vi "Test Remove Project.vi"(8 "error in (no error)":errorcluster, 10 "Work Folder":path, 11 "Test Data Folder":path) -> (0 "error out":errorcluster, 2 "Report":string, 3 "Passed":bool)   [LabVIEW 2024]
doc: "Removes the sample project \"Client Website\" with Project Store-INI, writes, and reads the files again into a NEW store: the project and all its tasks must be gone from memory and from disk, and the other projects must still be there.\n\nInputs: Test Data Folder holds the source copies (Samples, v1); each run works in a new case folder under Work Folder. Passed is TRUE when every check passed and no error occurred; Report lists every check.\n\nGenerated by: Claude"
uses:
  Storage/Project Store-INI/Project Store-INI.lvclass
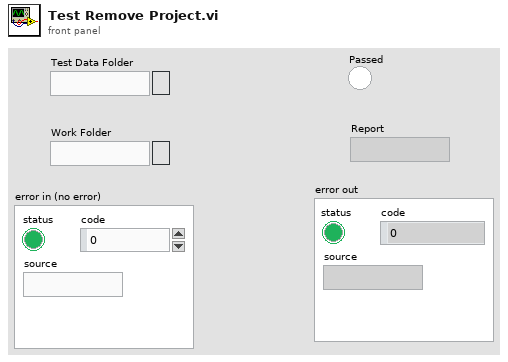
[diagram p1: front panel]
types:
  T1 = typedef "Task List.ctl" = T2[]
  T2 = typedef "Task.ctl" = cluster{"ID":string, "Project ID":string, "Name":string, "Active":bool, "Sort Order":i32}
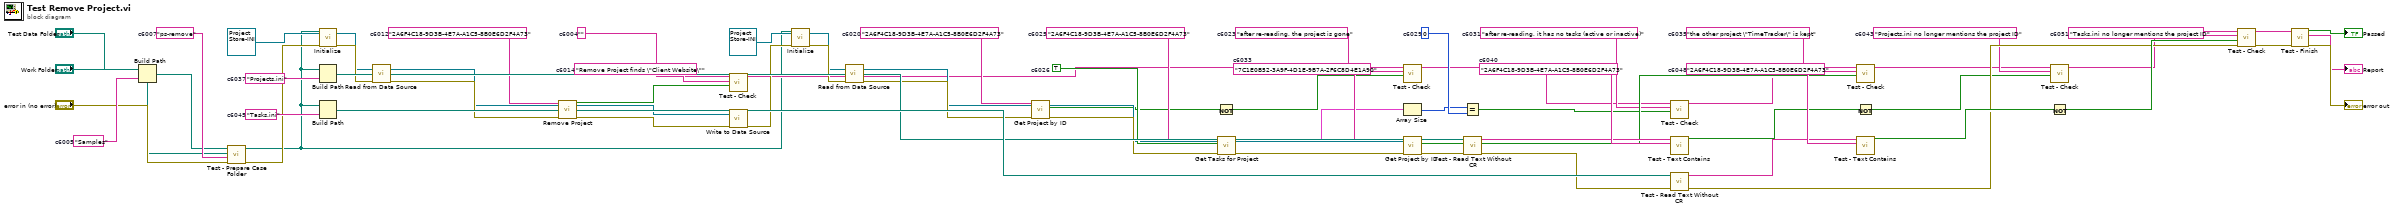
[diagram p0: block diagram]
diagram:
  w65 = "Tasks.ini no longer mentions the project ID"  # c6051
  w62 = "2A6F4C18-9D3B-4E7A-A1C5-8B0E6D2F4A73"  # c6048
  w58 = "Tasks.ini"  # c6045
  w56 = "Projects.ini no longer mentions the project ID"  # c6043
  w53 = "2A6F4C18-9D3B-4E7A-A1C5-8B0E6D2F4A73"  # c6040
  w49 = "Projects.ini"  # c6037
  w47 = "the other project \"TimeTracker\" is kept"  # c6035
  w44 = "7C1E0B52-3A9F-4D1E-9B7A-2F6C8D4E1A90"  # c6033
  w42 = "after re-reading, it has no tasks (active or inactive)"  # c6031
  w40 = 0  # c6029
  w35 = TRUE  # c6026
  w34 = "2A6F4C18-9D3B-4E7A-A1C5-8B0E6D2F4A73"  # c6025
  w32 = "after re-reading, the project is gone"  # c6023
  w27 = "2A6F4C18-9D3B-4E7A-A1C5-8B0E6D2F4A73"  # c6020
  w19 = "Remove Project finds \"Client Website\""  # c6014
  w15 = "2A6F4C18-9D3B-4E7A-A1C5-8B0E6D2F4A73"  # c6012
  w7 = "ps-remove"  # c6007
  w5 = "Samples"  # c6005
  w4 = ""  # c6004
  n1 = Build Path(base path="Test Data Folder", name or relative path=w5) -> (appended path=w6:path)
  n2 = call "Test - Prepare Case Folder.vi"("error in (no error)"="error in (no error)", "Case Name"=w7, "Work Folder"="Work Folder", "Source Folder"=w6) -> ("error out"=w9:errorcluster, "Case Folder"=w8:path)  [unwired: 6 in]
  n3 = call-dynamic "Initialize.vi"("Project Store in"=refnum<class "Project Store-INI.lvclass"> refnum ("Project Store-INI"), "error in (no error)"=w9, "Data Folder"=w8) -> ("error out"=w12:errorcluster, "Project Store out"=w11:refnum<class "Project Store-INI.lvclass">)  [unwired: 7 in]
  n4 = Build Path(base path=w8, name or relative path=w49) -> (appended path=w50:path)
  n5 = Build Path(base path=w8, name or relative path=w58) -> (appended path=w59:path)
  n6 = call-dynamic "Read from Data Source.vi"("Project Store in"=w11, "error in (no error)"=w12) -> ("error out"=w14:errorcluster, "Project Store out"=w13:refnum<class "Project Store-INI.lvclass">)  [unwired: 8 in]
  n7 = call-dynamic "Remove Project.vi"("Project Store in"=w13, "error in (no error)"=w14, "ID"=w15) -> ("error out"=w18:errorcluster, "found?"=w16:bool, "Project Store out"=w17:refnum<class "Project Store-INI.lvclass">)  [unwired: 6 in]
  n8 = call "Test - Check.vi"("Condition"=w16, "Check Name"=w19, "Report in"=w4) -> ("Report out"=w20:string)  [unwired: 7 in, 1 out]
  n9 = call-dynamic "Write to Data Source.vi"("Project Store in"=w17, "error in (no error)"=w18) -> ("error out"=w21:errorcluster)  [unwired: 8 in, 1 out]
  n10 = call-dynamic "Initialize.vi"("Project Store in"=refnum<class "Project Store-INI.lvclass"> refnum ("Project Store-INI"), "error in (no error)"=w21, "Data Folder"=w8) -> ("error out"=w24:errorcluster, "Project Store out"=w23:refnum<class "Project Store-INI.lvclass">)  [unwired: 7 in]
  n11 = call-dynamic "Read from Data Source.vi"("Project Store in"=w23, "error in (no error)"=w24) -> ("error out"=w26:errorcluster, "Project Store out"=w25:refnum<class "Project Store-INI.lvclass">)  [unwired: 8 in]
  n12 = call-dynamic "Get Project by ID.vi"("Project Store in"=w25, "error in (no error)"=w26, "ID"=w27) -> ("error out"=w30:errorcluster, "found?"=w28:bool, "Project Store out"=w29:refnum<class "Project Store-INI.lvclass">)  [unwired: 5 in, 1 out]
  n13 = Not(x=w28) -> (.not. x?=w31:bool)
  n14 = call-dynamic "Get Tasks for Project.vi"("Project Store in"=w29, "error in (no error)"=w30, "include inactive?"=w35, "Project ID"=w34) -> ("error out"=w38:errorcluster, "Tasks"=w36:T1, "Project Store out"=w37:refnum<class "Project Store-INI.lvclass">)  [unwired: 5 in]
  n15 = call "Test - Check.vi"("Condition"=w31, "Check Name"=w32, "Report in"=w20) -> ("Report out"=w33:string)  [unwired: 7 in, 1 out]
  n16 = Array Size(array=w36) -> (size(s)=w39:i32)
  n17 = call-dynamic "Get Project by ID.vi"("Project Store in"=w37, "error in (no error)"=w38, "ID"=w44) -> ("error out"=w46:errorcluster, "found?"=w45:bool)  [unwired: 5 in, 2 out]
  n18 = Equal?(x=w39, y=w40) -> (x = y?=w41:bool)
  n19 = call "Test - Read Text Without CR.vi"("error in (no error)"=w46, "File"=w50) -> ("error out"=w52:errorcluster, "Text"=w51:string)  [unwired: 8 in]
  n20 = call "Test - Check.vi"("Condition"=w41, "Check Name"=w42, "Report in"=w33) -> ("Report out"=w43:string)  [unwired: 7 in, 1 out]
  n21 = call "Test - Text Contains.vi"("Search Text"=w53, "Text"=w51) -> ("Contains?"=w54:bool)  [unwired: 8 in, 1 out]
  n22 = call "Test - Read Text Without CR.vi"("error in (no error)"=w52, "File"=w59) -> ("error out"=w61:errorcluster, "Text"=w60:string)  [unwired: 8 in]
  n23 = call "Test - Check.vi"("Condition"=w45, "Check Name"=w47, "Report in"=w43) -> ("Report out"=w48:string)  [unwired: 7 in, 1 out]
  n24 = Not(x=w54) -> (.not. x?=w55:bool)
  n25 = call "Test - Text Contains.vi"("Search Text"=w62, "Text"=w60) -> ("Contains?"=w63:bool)  [unwired: 8 in, 1 out]
  n26 = call "Test - Check.vi"("Condition"=w55, "Check Name"=w56, "Report in"=w48) -> ("Report out"=w57:string)  [unwired: 7 in, 1 out]
  n27 = Not(x=w63) -> (.not. x?=w64:bool)
  n28 = call "Test - Check.vi"("Condition"=w64, "Check Name"=w65, "Report in"=w57) -> ("Report out"=w66:string)  [unwired: 7 in, 1 out]
  n29 = call "Test - Finish.vi"("error in (no error)"=w61, "Report"=w66) -> ("error out"=→"error out":errorcluster, "Report out"=→"Report":string, "Passed"=→"Passed":bool)  [unwired: 7 in]
